vi "_Subsystem_Name Controller.vi"(8 "error in":errorcluster) -> ()   [LabVIEW 2023]
doc: "This VI responds to drive commands both auto and tele Opmodes.\nIt owns the drivebase motors and sensors and runs independent from opModes. Commands can run for arbitrary times, but newly posted commands will interupt as long as Check is called and used for time delays."
uses:
  _Subsystem_Name Operations.ctl
  _Subsystem_Name Setpoints.ctl
  <vilib>/MRC/Types/CmdCtl Completion.ctl
  <vilib>/Rock Robotics/WPI/Framework/Completion Status.ctl
panel:
  in  "Abort Cmd":bool
  in  "Execute Cmd":bool
  in  "Interactive Values":T1
  out "Command Timing":cluster{"Start Time (ms)":u32, "Iterations":i32}
  out "Status":T3
  out "Current Command Data":T1
  out "Cmd Summary":string
  # "Interactive Command: You may fill in the settings for a command\nand schedule it with the Execute button. You can observe and abort\nany command while fine tuning the code for the controller."
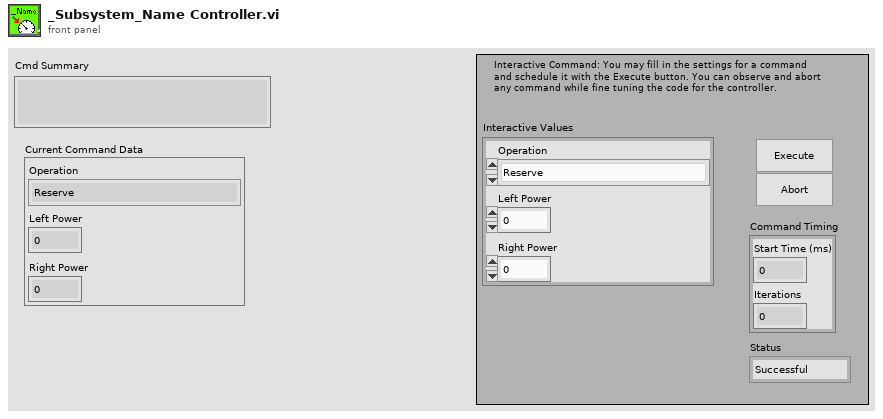
[diagram p1: front panel]
types:
  T1 = typedef "_Subsystem_Name Setpoints.ctl" = cluster{"Operation":T2, "Left Power":dbl, "Right Power":dbl}
  T2 = typedef "_Subsystem_Name Operations.ctl" = enum16{"Reserve", "Read Current", "Immediate"}
  T3 = typedef "Completion Status.ctl" = enum16{"Successful", "Aborted", "Incomplete"}
  T4 = typedef "Command Status Info.ctl" = cluster{"Name":string, "Status":T3, "notifier out":T5}
  T5 = typedef "Completion Notifier.ctl" = refnum<notifier>
  T6 = cluster{"Current Command":T1, "Command Timing":cluster{"Start Time (ms)":u32, "Iterations":i32}, "Command Arguments":cluster{"Command Info":T4, "Description":string, "Default Command":T1, "queue out":refnum<queue>, "Subsystem Name":string}}
  T7 = typedef "CmdCtl Completion.ctl" = enum16{"incomplete", "finished"}
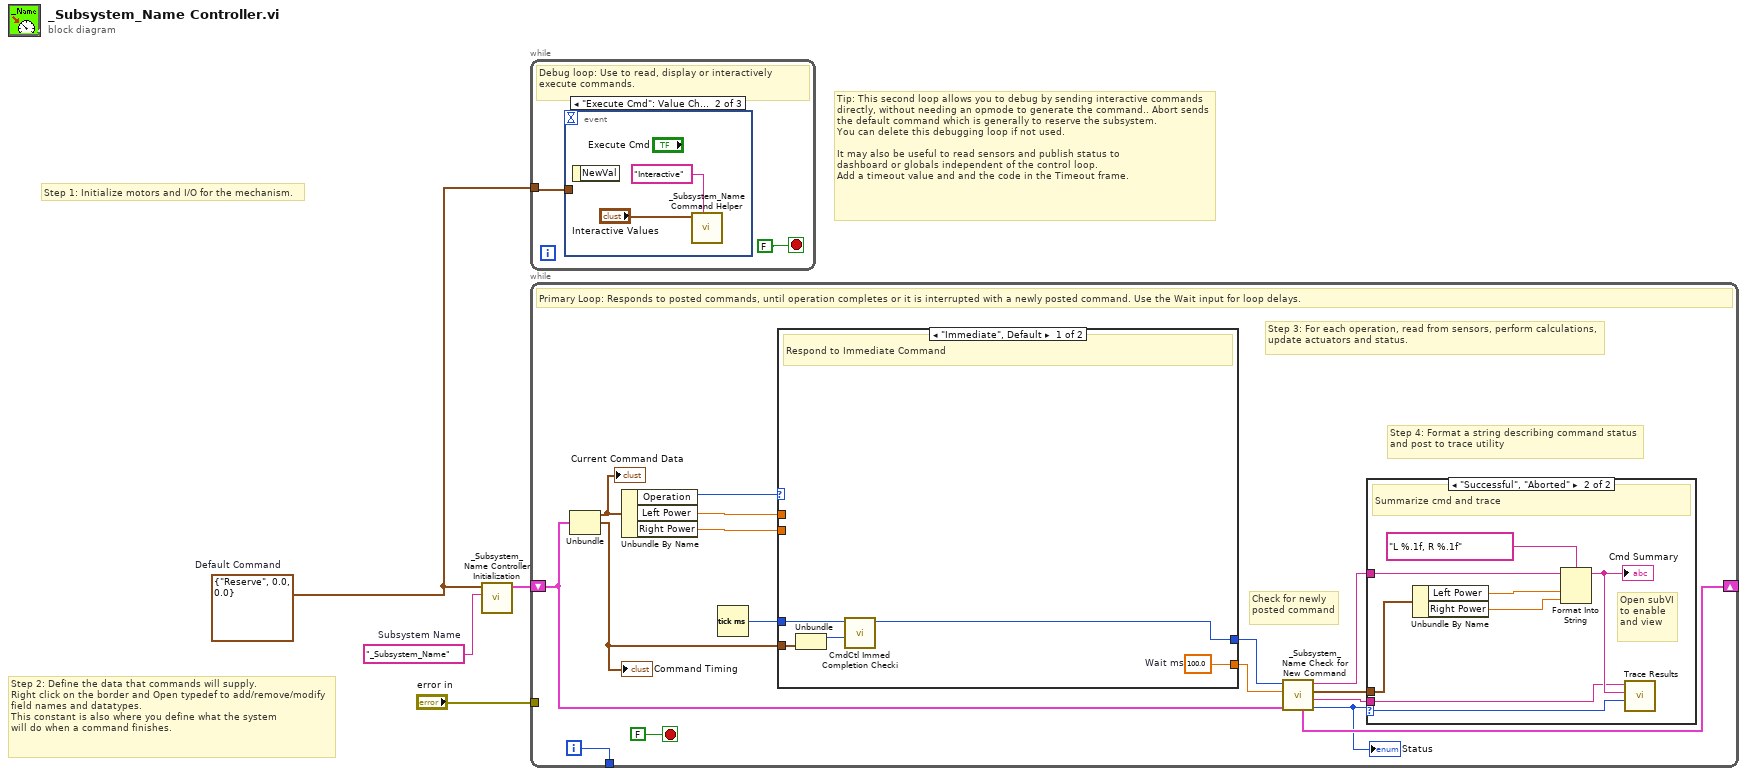
[diagram p0: block diagram]
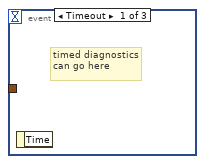
[diagram p2: hidden frame]
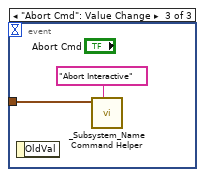
[diagram p3: hidden frame]
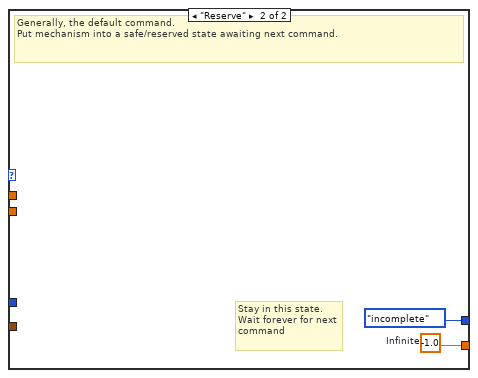
[diagram p5: hidden frame]
diagram:
  w1 = T1 {"Operation"=enum."Reserve", "Left Power"=0.0, "Right Power"=0.0}  # Default Command
  w2 = "_Subsystem_Name"  # Subsystem Name
  # "Tip: This second loop allows you to debug by sending interactive commands\ndirectly, without needing an opmode to generate the command.. Abort sends\nthe default command which is generally to reserve the subsystem.\nYou can delete this debugging loop if not used.\n\nIt may also be useful to read sensors and publish status to\ndashboard or globals independent of the control loop.\nAdd a timeout value and and the code in the Timeout frame."
  # "Step 2: Define the data that commands will supply.\nRight click on the border and Open typedef to add/remove/modify\nfield names and datatypes.\nThis constant is also where you define what the system\nwill do when a command finishes."
  # "Step 1: Initialize motors and I/O for the mechanism."
  n1 = call "_Subsystem_Name Controller Initialization.vi"("Subsystem Name"=w2, "Default Command"=w1) -> ("Current Command"=w3:T6)  [unwired: 9 in]
  n2 = while {
    tunnel: w1 -> [w5]
    stop <- FALSE stop-if-true
    # "Debug loop: Use to read, display or interactively execute commands."
    n3 = event shown="[1] \"Execute Cmd\": Value Change" {
      selector: _ -> [_ _ _]
      dyn-events: _ -> [_ _ _]
      timeout: _ -> [_ _ _]
      tunnel: w5 -> [_ _ w10]
      event Timeout {
        # "timed diagnostics\ncan go here"
        # "Insert Text Here"
        n4 = event-data() -> ()  [unwired: 1 in, 1 out]
      }
      event "Execute Cmd": Value Change {
        # "Execute"
        n5 = event-data() -> ()  [unwired: 1 in, 1 out]
        n6 = call "_Subsystem_Name Command Helper.vi"("Description"="Interactive", "SubSystem Data"="Interactive Values") -> ()  [unwired: 7 in, 3 out]
      }
      event "Abort Cmd": Value Change {
        # "Insert Text Here"
        n7 = event-data() -> ()  [unwired: 1 in, 1 out]
        n8 = call "_Subsystem_Name Command Helper.vi"("Description"="Abort Interactive", "SubSystem Data"=w10) -> ()  [unwired: 7 in, 3 out]
      }
    }
  }
  n9 = while {
    shift-right: [w20] -> _
    shift-left: w3 -> [w14]
    tunnel: [w25] -> _
    tunnel: "error in" -> [_]
    i -> [w25]
    stop <- FALSE stop-if-true
    # "Step 4: Format a string describing command status\nand post to trace utility"
    # "Check for newly\nposted command"
    # "Step 3: For each operation, read from sensors, perform calculations,\nupdate actuators and status."
    # "Primary Loop: Responds to posted commands, until operation completes or it is interrupted with a newly posted command. Use the Wait input for loop delays."
    n10 = Unbundle(w14) -> ("Current Command"=w12:T1, "Command Timing"=w13:cluster{"Start Time (ms)":u32, "Iterations":i32})  [unwired: 1 out]
    "Command Timing" <- w13
    "Current Command Data" <- w12
    n11 = Unbundle By Name(w12) -> ("Operation"=w24:T2, "Left Power"=w23:dbl, "Right Power"=w21:dbl)
    n12 = Tick Count (ms)() -> (millisecond timer value=w22:u32)
    n13 = case shown="\"Immediate\", Default" w24 {
      tunnel: [w39 w41] -> w18
      tunnel: [w36 CmdCtl_Completion."incomplete"] -> w19
      tunnel: w13 -> [w38 _]
      tunnel: w23 -> [_ _]
      tunnel: w22 -> [w37 _]
      tunnel: w21 -> [_ _]
      frame "Immediate", Default {
        w39 = 100.0  # Wait ms
        # "Respond to Immediate Command"
        n14 = Unbundle(w38) -> ("Start Time (ms)"=w35:u32)  [unwired: 1 out]
        n15 = call <vilib>:"CmdCtl Immed Completion Checki.vi"("Start Time (ms)"=w35, "current time (ms)"=w37) -> ("Completion"=w36:T7)  [unwired: 9 in]
      }
      frame "Reserve" {
        w41 = -1.0  # Infinite
        # "Stay in this state.\nWait forever for next\ncommand"
        # "Generally, the default command.\nPut mechanism into a safe/reserved state awaiting next command."
      }
    }
    n16 = call "_Subsystem_Name Check for New Command.vi"("Current Command"=w14, "Wait time (ms)"=w18, "Completion"=w19) -> ("Completion"=w11:T3, "Subsystem Name"=w15:string, "Current Command"=w16:T1, "Initial Trace String"=w17:string, "NextCommand"=w20:T6)  [unwired: 4 in]
    "Status" <- w11
    n17 = case shown="\"Successful\", \"Aborted\"" w11 {
      selector: w11 -> [_ w34]
      tunnel: w17 -> [_ w30]
      tunnel: w16 -> [_ w31]
      tunnel: w15 -> [_ w27]
      frame "Incomplete", Default {
        # "Continuing current command"
      }
      frame "Successful", "Aborted" {
        # "Open subVI\nto enable\nand view"
        # "Summarize cmd and trace"
        n18 = Unbundle By Name(w31) -> ("Left Power"=w33:dbl, "Right Power"=w28:dbl)
        n19 = Format Into String(format string="L %.1f, R %.1f", initial string=w30, w33, w28) -> (resulting string=w29:string)  [unwired: 1 in, 1 out]
        "Cmd Summary" <- w29
        n20 = call <vilib>:"Trace Results.vi"("Status of previous command"=w34, "Description"=w29, "Subsystem"=w27) -> ()  [unwired: 9 in]
      }
    }
  }
